vi "Run Test - Refine Data (SubVI) (1).vi"(0 "Sensor Data":sgl[](array[numeric]), 1 "Data In":sgl, 3 "index":i32) -> (4 "Data Out":dbl)   [LabVIEW 2019]
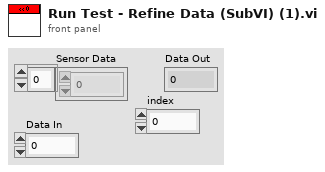
[diagram p1: front panel]
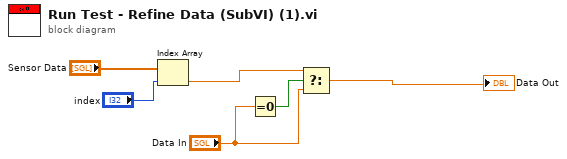
[diagram p0: block diagram]
diagram:
  n1 = Index Array(array="Sensor Data", index="index") -> (element=w6:sgl)
  n2 = Equal To 0?(x="Data In") -> (x = 0?=w3:bool)
  n3 = Select(t=w6, s=w3, f="Data In") -> (s? t:f=→"Data Out":sgl)
